vi "Position_Command.vi"(8 "error in (no error)":errorcluster, 10 "Elevator Position Control":dbl, 11 "Elevator in":refnum<class "Elevator.lvclass">) -> (0 "error out":errorcluster, 3 "Elevator out":refnum<class "Elevator.lvclass">)   [LabVIEW 2021, in "Elevator.lvclass"]
uses:
  Elevator.lvclass
  Elevator.lvclass/Elevator.ctl
  AnalogOutput/AnalogOutput.lvclass
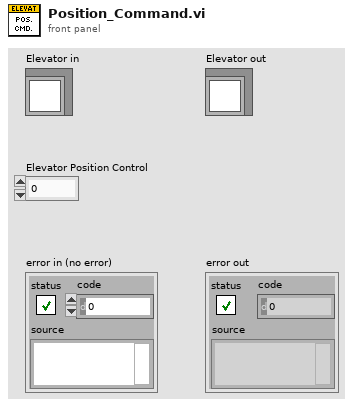
[diagram p1: front panel]
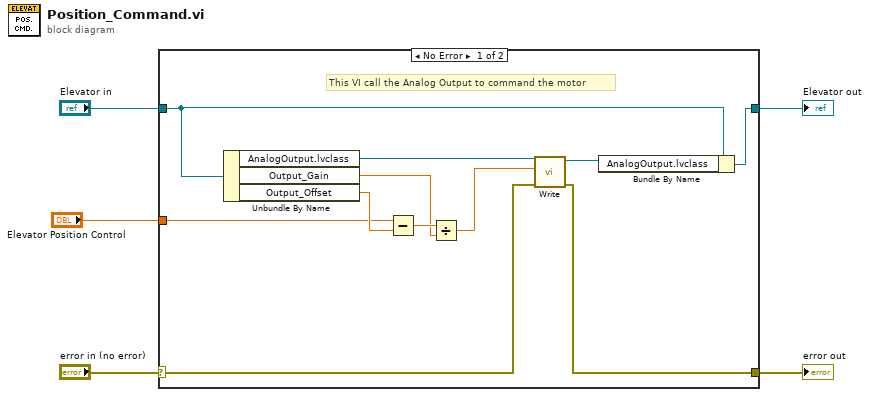
[diagram p0: block diagram]
diagram:
  n1 = case shown="No Error" "error in (no error)" {
    selector: "error in (no error)" -> [w15 w18]
    tunnel: [w14 w18] -> w2
    tunnel: [w11 w17] -> w3
    tunnel: "Elevator in" -> [w12 w17]
    tunnel: "Elevator Position Control" -> [w9 _]
    frame No Error {
      # "This VI call the Analog Output to command the motor"
      n2 = Unbundle By Name(w12) -> ("AnalogOutput.lvclass"=w16:refnum<class "AnalogOutput.lvclass">, "Output_Gain"=w7:dbl, "Output_Offset"=w10:dbl)
      n3 = Subtract(x=w9, y=w10) -> (x-y=w8:dbl)
      n4 = Divide(x=w8, y=w7) -> (x/y=w6:dbl)
      n5 = call-dynamic "Write.vi"("error in (no error)"=w15, "data in"=w6, "AnalogOutput in"=w16) -> ("error out"=w14:errorcluster, "AnalogOutput out"=w13:refnum<class "AnalogOutput.lvclass">)  [unwired: 7 in]
      n6 = Bundle By Name(cluster=w12, "AnalogOutput.lvclass"=w13) -> (w11:refnum<class "Elevator.lvclass">)
    }
    frame Error {
    }
  }
  "error out" <- w2
  "Elevator out" <- w3
